vi "4Pi Dual DM - Make Mirror Pattern.vi"(0 "Mirror Modes In":T1, 2 "Flat On?":bool, 7 "Flat File In":dbl[](array[numeric]), 11 "Mirror Modes Array":dbl[][](array[numeric])) -> (8 "Pixel Value U (-1 to 1)":dbl[](array[numeric]))   [LabVIEW 2021]
uses:
  4Pi Dual DM - Controls/4Pi Dual DM - Mirror Modes.ctl
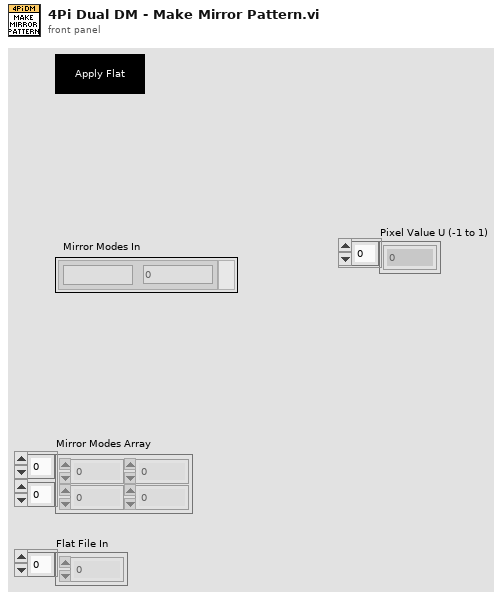
[diagram p1: front panel]
types:
  T1 = typedef "4Pi Dual DM - Mirror Modes.ctl" = cluster{"Mode":string, "Amplitude":dbl}[]
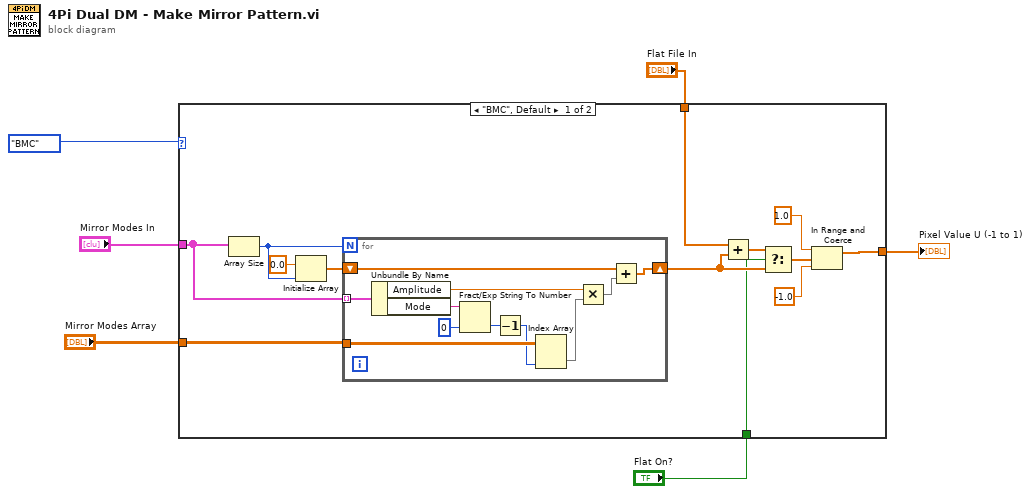
[diagram p0: block diagram]
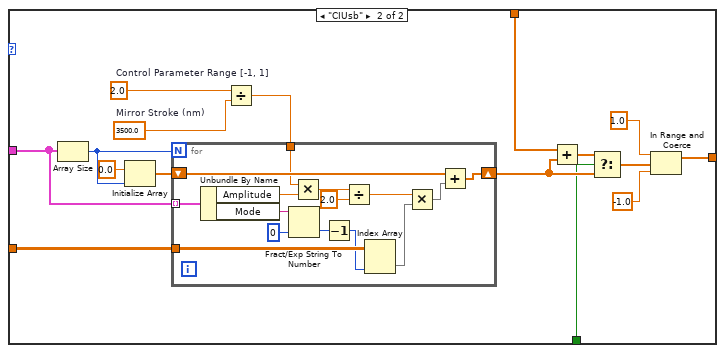
[diagram p2: hidden frame]
diagram:
  n1 = case shown="\"BMC\", Default" enum16{"BMC", "CIUsb"}."BMC" {
    tunnel: "Mirror Modes In" -> [w11 w38]
    tunnel: "Mirror Modes Array" -> [w14 w37]
    tunnel: "Flat On?" -> [w13 w36]
    tunnel: "Flat File In" -> [w12 w35]
    tunnel: [w7 w31] -> w1
    frame "BMC", Default {
      n2 = Array Size(array=w11) -> (size(s)=w16:i32)
      n3 = Initialize Array(0.0 ("element"), w16) -> (w19:dbl[])
      n4 = for {
        N: w16 -> [_]
        tunnel: w11 -> [w30] mode=indexing
        shift-right: [w23] -> w18
        shift-left: w19 -> [w24]
        tunnel: w14 -> [w26]
        n5 = Unbundle By Name(w30) -> ("Amplitude"=w20:dbl, "Mode"=w28:string)
        n6 = Fract/Exp String To Number(string=w28, default (0 dbl)=0) -> (number=w27:i32)  [unwired: 2 in, 1 out]
        n7 = Decrement(x=w27) -> (x-1=w25:i32)
        n8 = Index Array(array=w26, index (col)=w25) -> (element=w21:dbl[])  [unwired: 1 in]
        n9 = Multiply(x=w20, y=w21) -> (x*y=w22:dbl[])
        n10 = Add(x=w24, y=w22) -> (x+y=w23:dbl[])
      }
      n11 = Add(x=w12, y=w18) -> (x+y=w17:dbl[])
      n12 = Select(t=w17, s=w13, f=w18) -> (s? t:f=w10:dbl[])
      n13 = In Range and Coerce(upper limit=1.0, x=w10, lower limit=-1.0) -> (coerced(x)=w7:dbl[])  [unwired: 1 out]
    }
    frame "CIUsb" {
      w44 = 3500.0  # Mirror Stroke (nm)
      w43 = 2.0  # Control Parameter Range [-1, 1]
      n14 = Array Size(array=w38) -> (size(s)=w45:i32)
      n15 = Initialize Array(0.0 ("element"), w45) -> (w39:dbl[])
      n16 = Divide(x=w43, y=w44) -> (x/y=w42:dbl)
      n17 = for {
        N: w45 -> [_]
        tunnel: w38 -> [w61] mode=indexing
        shift-right: [w54] -> w40
        shift-left: w39 -> [w55]
        tunnel: w37 -> [w57]
        tunnel: w42 -> [w48]
        n18 = Unbundle By Name(w61) -> ("Amplitude"=w49:dbl, "Mode"=w59:string)
        n19 = Fract/Exp String To Number(string=w59, default (0 dbl)=0) -> (number=w58:i32)  [unwired: 2 in, 1 out]
        n20 = Multiply(x=w48, y=w49) -> (x*y=w51:dbl)
        n21 = Decrement(x=w58) -> (x-1=w56:i32)
        n22 = Divide(x=w51, y=2.0) -> (x/y=w50:dbl)
        n23 = Index Array(array=w57, index (col)=w56) -> (element=w47:dbl[])  [unwired: 1 in]
        n24 = Multiply(x=w50, y=w47) -> (x*y=w53:dbl[])
        n25 = Add(x=w55, y=w53) -> (x+y=w54:dbl[])
      }
      n26 = Add(x=w35, y=w40) -> (x+y=w41:dbl[])
      n27 = Select(t=w41, s=w36, f=w40) -> (s? t:f=w32:dbl[])
      n28 = In Range and Coerce(upper limit=1.0, x=w32, lower limit=-1.0) -> (coerced(x)=w31:dbl[])  [unwired: 1 out]
    }
  }
  "Pixel Value U (-1 to 1)" <- w1
